vi "VI Helpeks Website.vi"   [LabVIEW 2014]
doc: "::: VI Helpeks :::\nCopyright (c) 2000-2026 Konstantin Shifershteyn. All rights reserved."
uses:
  <vilib>/Platform/browser.llb/Open URL in Default Browser (string).vi
panel:
  # "VI Helpeks Website"
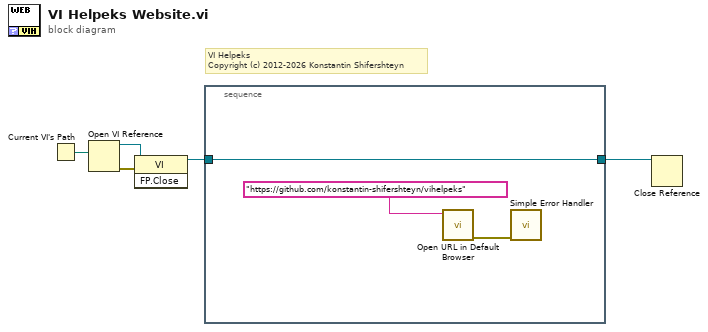
[diagram p0: block diagram]
diagram:
  # "VI Helpeks\nCopyright (c) 2012-2026 Konstantin Shifershteyn"
  n1 = Current VI's Path() -> (path=w1:path)
  n2 = Open VI Reference(vi path=w1) -> (vi reference=w4:refnum<vi>, error out=w5:errorcluster)  [unwired: 5 in]
  n3 = invoke class="VI" method="FP.Close"(reference=w4, error in=w5) -> (reference out=w3:refnum<vi>)  [unwired: 1 in, 2 out]
  n4 = stacked-sequence {
    tunnel: [w8] -> w2
    tunnel: w3 -> [w8]
    frame #0 {
      n5 = call-poly <vilib>:"Open URL in Default Browser.vi"("URL"="https://github.com/konstantin-shifershteyn/vihelpeks") -> ("error out"=w6:errorcluster)  [unwired: 5 in, 1 out]
      n6 = call <vilib>:"Simple Error Handler.vi"("error in (no error)"=w6) -> ()  [unwired: 4 in, 5 out]
    }
  }
  n7 = Close Reference(reference=w2) -> ()  [unwired: 1 in, 1 out]
